vi "Lock Displays AE.vi"(0 "Lock All Markers":bool, 2 "Action":T1, 7 "Lock All AutoScale":bool, 9 "Show All Z Scale":bool, 11 "Lock Pan/Zoom":bool) -> (4 "Lock All Markers Out":bool, 8 "Lock All AutoScale Out":bool, 10 "Show All Z Scale Out":bool, 15 "Lock Pan/Zoom Out":bool)   [LabVIEW 2021]
uses:
  Hardware Configuration/Hardware Configuration Controls/Standard Action.ctl
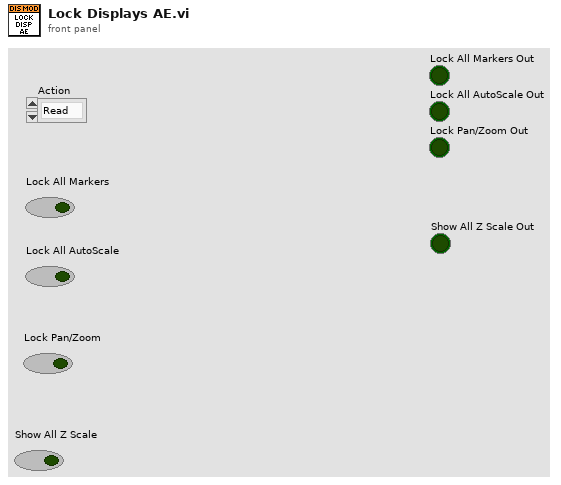
[diagram p1: front panel]
types:
  T1 = typedef "Standard Action.ctl" = enum16{"Read", "Write"}
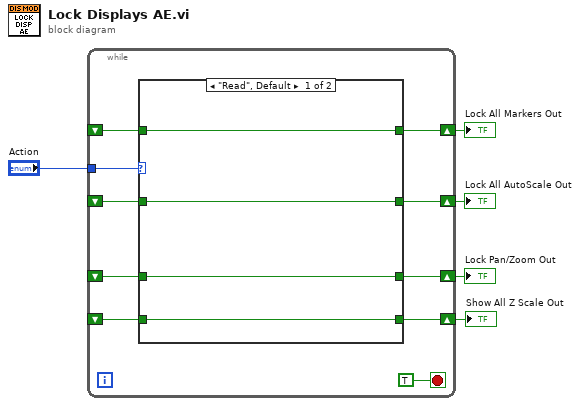
[diagram p0: block diagram]
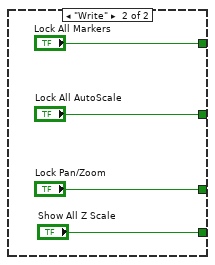
[diagram p2: hidden frame]
diagram:
  n1 = while {
    shift-right: [w13] -> w4
    shift-left: _ -> [w10]
    shift-right: [w12] -> w3
    shift-left: _ -> [w9]
    shift-right: [w11] -> w2
    shift-left: _ -> [w8]
    tunnel: "Action" -> [w14]
    shift-right: [w7] -> w1
    shift-left: _ -> [w6]
    stop <- TRUE stop-if-true
    n2 = case shown="\"Read\", Default" w14 {
      tunnel: [w19 "Lock All Markers"] -> w13
      tunnel: [w18 "Lock All AutoScale"] -> w12
      tunnel: [w17 "Lock Pan/Zoom"] -> w11
      tunnel: w10 -> [w19 _]
      tunnel: w9 -> [w18 _]
      tunnel: w8 -> [w17 _]
      tunnel: [w16 "Show All Z Scale"] -> w7
      tunnel: w6 -> [w16 _]
      frame "Read", Default {
      }
      frame "Write" {
      }
    }
  }
  "Lock All Markers Out" <- w4
  "Lock All AutoScale Out" <- w3
  "Lock Pan/Zoom Out" <- w2
  "Show All Z Scale Out" <- w1
